vi "test_input_required_result_prompt.vi"(8 "error in":errorcluster) -> (0 "error out":errorcluster, 3 "prompt":string)   [LabVIEW 2020, in "Conformance MCP Server.lvlib"]
doc: "Conformance fixture (scenario input-required-result-non-tool-request). A prompt without arguments that asks the user \"What context should the prompt use?\" with Ask User.vi (key user_context, a form with the string context) and returns the text \"Use this context: <context>\". Without an accepted answer it returns at once with the text \"No context was given.\""
uses:
  Conformance MCP Server.lvlib
  <vilib>/JDP Science/JSONtext/Next JSON Value.vi
  <vilib>/JDP Science/JSONtext/String Subset.vi
  <vilib>/JDP Science/JSONtext/support/Strip Quotes and Unescape.vi
  <vilib>/JDP Science/JSONtext/Parsing/Advance past next JSON Value (inlined COPY).vi
  <vilib>/JDP Science/JSONtext/support/Unescape JSON string.vi
  <vilib>/JDP Science/JSONtext/Parsing/Advance past whitespace.vi
  <vilib>/JDP Science/JSONtext/Parsing/Advance past String.vi
  <vilib>/JDP Science/JSONtext/Parsing/Advance past Number.vi
  <vilib>/JDP Science/JSONtext/Parsing/Advance past Line Ending.vi
  <vilib>/JDP Science/JSONtext/Parsing/Parse Full Path or Item Name.vi
  <vilib>/JDP Science/JSONtext/Parsing/Advance past Array.vi
  <vilib>/JDP Science/JSONtext/Parsing/Advance past Object.vi
  <vilib>/JDP Science/JSONtext/support/Error Cluster From Code.vi
  <vilib>/JDP Science/JSONtext/Offset/Find Item Locations by Path.vi
  <vilib>/JDP Science/JSONtext/Parsing/Advance past next JSON Value.vi
  src/MCP Server/MCP Server.lvlib
  <vilib>/JDP Science/JSONtext/JSONtext.lvlib
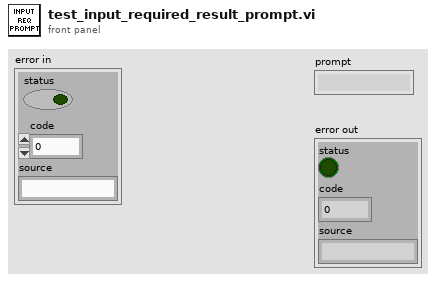
[diagram p1: front panel]
types:
  T1 = enum16{"accept", "decline", "cancel", "pending", "not supported"}
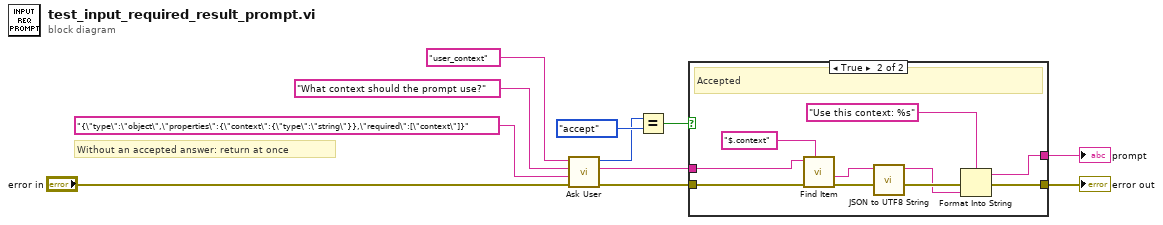
[diagram p0: block diagram]
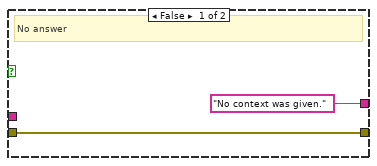
[diagram p2: hidden frame]
diagram:
  # "Without an accepted answer: return at once"
  n1 = call "Ask User.vi"("error in"="error in", "requestedSchema"="{\"type\":\"object\",\"properties\":{\"context\":{\"type\":\"string\"}},\"required\":[\"context\"]}", "message"="What context should the prompt use?", "key"="user_context") -> ("error out"=w7:errorcluster, "content"=w6:string, "action"=w5:T1)  [unwired: 5 in]
  n2 = Equal?(x=w5, y=T1."accept" ("accept")) -> (x = y?=w9:bool)
  n3 = case shown="True" w9 {
    tunnel: w6 -> [_ w14]
    tunnel: w7 -> [w12 w15]
    tunnel: ["No context was given." ("text") w22] -> w10
    tunnel: [w12 w23] -> w11
    frame False {
      # "No answer"
    }
    frame True {
      # "Accepted"
      n4 = call <vilib>:"Find Item.vi"("$Path or Item Name"="$.context", "error in (no error)"=w15, "JSON"=w14) -> ("error out"=w17:errorcluster, "<JSON>"=w18:string)  [unwired: 5 in, 2 out]
      n5 = call <vilib>:"JSON to UTF8 String.vi"("error in (no error)"=w17, "JSON"=w18) -> ("error out"=w20:errorcluster, "<UTF8>String"=w19:string)  [unwired: 8 in]
      n6 = Format Into String(format string="Use this context: %s", error in=w20, w19) -> (resulting string=w22:string, error out=w23:errorcluster)  [unwired: 1 in]
    }
  }
  "prompt" <- w10
  "error out" <- w11
